vi "FileCreatorMain.vi"() -> ()   [LabVIEW 2017]
uses:
  AutoFileDataType.ctl
panel:
  in  "Flip This Auto":bool
  in  "Auto":T1
  in  "Path File Name":string[](array[string])
  out "standard output":string
  out "standard error":string="NI Linux Real-Time (run mode)\n\nLog in with your NI-Auth credentials.\n\n"
  in  "ExportAllToRobot":bool
  in  "SaveToLocal":bool
  in  "LoadFromLocal":bool
  in  "ExportToRobot":bool
  in  "LoadAllFromRobot":bool
  in  "LocalFiles":i32(listbox)=2
  in  "LocalFileNames":string[](array[string])=["1A.txt", "1B.txt", "1C.txt", "1D.txt", "2A.txt", "2B.txt", "2C.txt", "2D.txt", "3A.txt", "3B.txt", "3C.txt", "3D.txt", "4A.txt", "4B.txt", "4C.txt", "4D.txt"]
  # "Drive:\nWait or\nStart"
  # "Elevator:\nWait or\nStart"
  # "Intake:\nWait or\nStart"
  # "Distance \nfor\nElevator"
  # "Degrees \nto turn"
  # "Elevator\nCommand"
  # "Time for \nintake"
  # "Drive\ncommand"
  # "Time\nfor elevator"
  # "Elevator\n Speed"
  # "Intake \nCommand"
  # "Path File Path"
  # "Speed"
  # "Distance(in)"
  # "Intake Speed"
  # "Drive commands:\n1. For time\n2. For distance\n3. Turn for angle\n4. Stop\n5. Drive Path\n6. Turn To Angle\n7. Drive to Cube"
  # "Elevator Commands:\n1. For time\n2. To distance\n3. Stop\n4. Pause for time, then distance"
  # "Intake Commands:\n1. For time\n2. Until cube\n3. Stop"
  # "Wait: 0\nStart: 1"
  # "Responses of CMDs run"
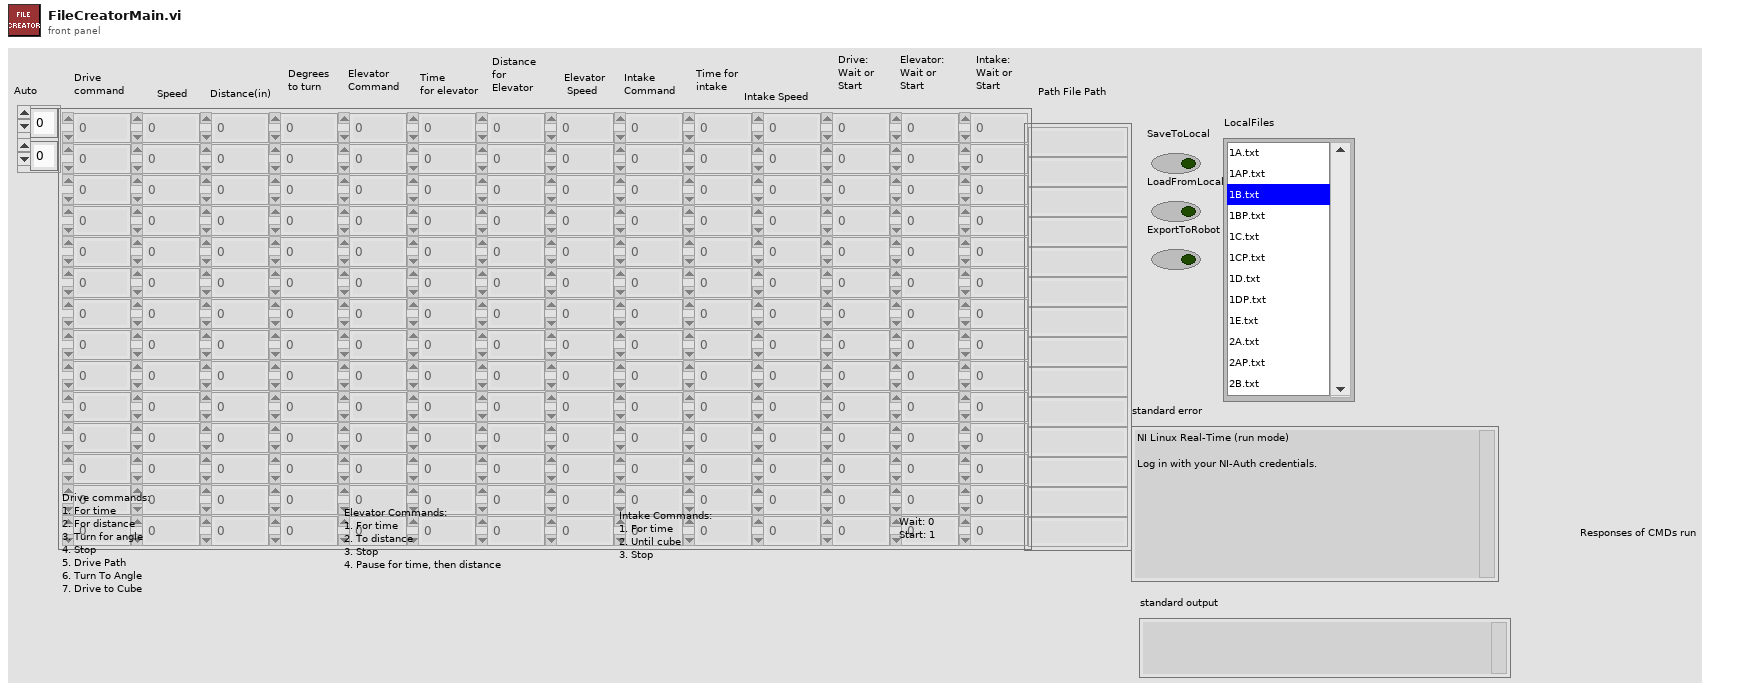
[diagram p1: front panel]
types:
  T1 = typedef "AutoFileDataType.ctl" = dbl[][]
  T2 = enum16{"open", "replace", "create", "open or create", "replace or create", "replace or create with confirmation"}
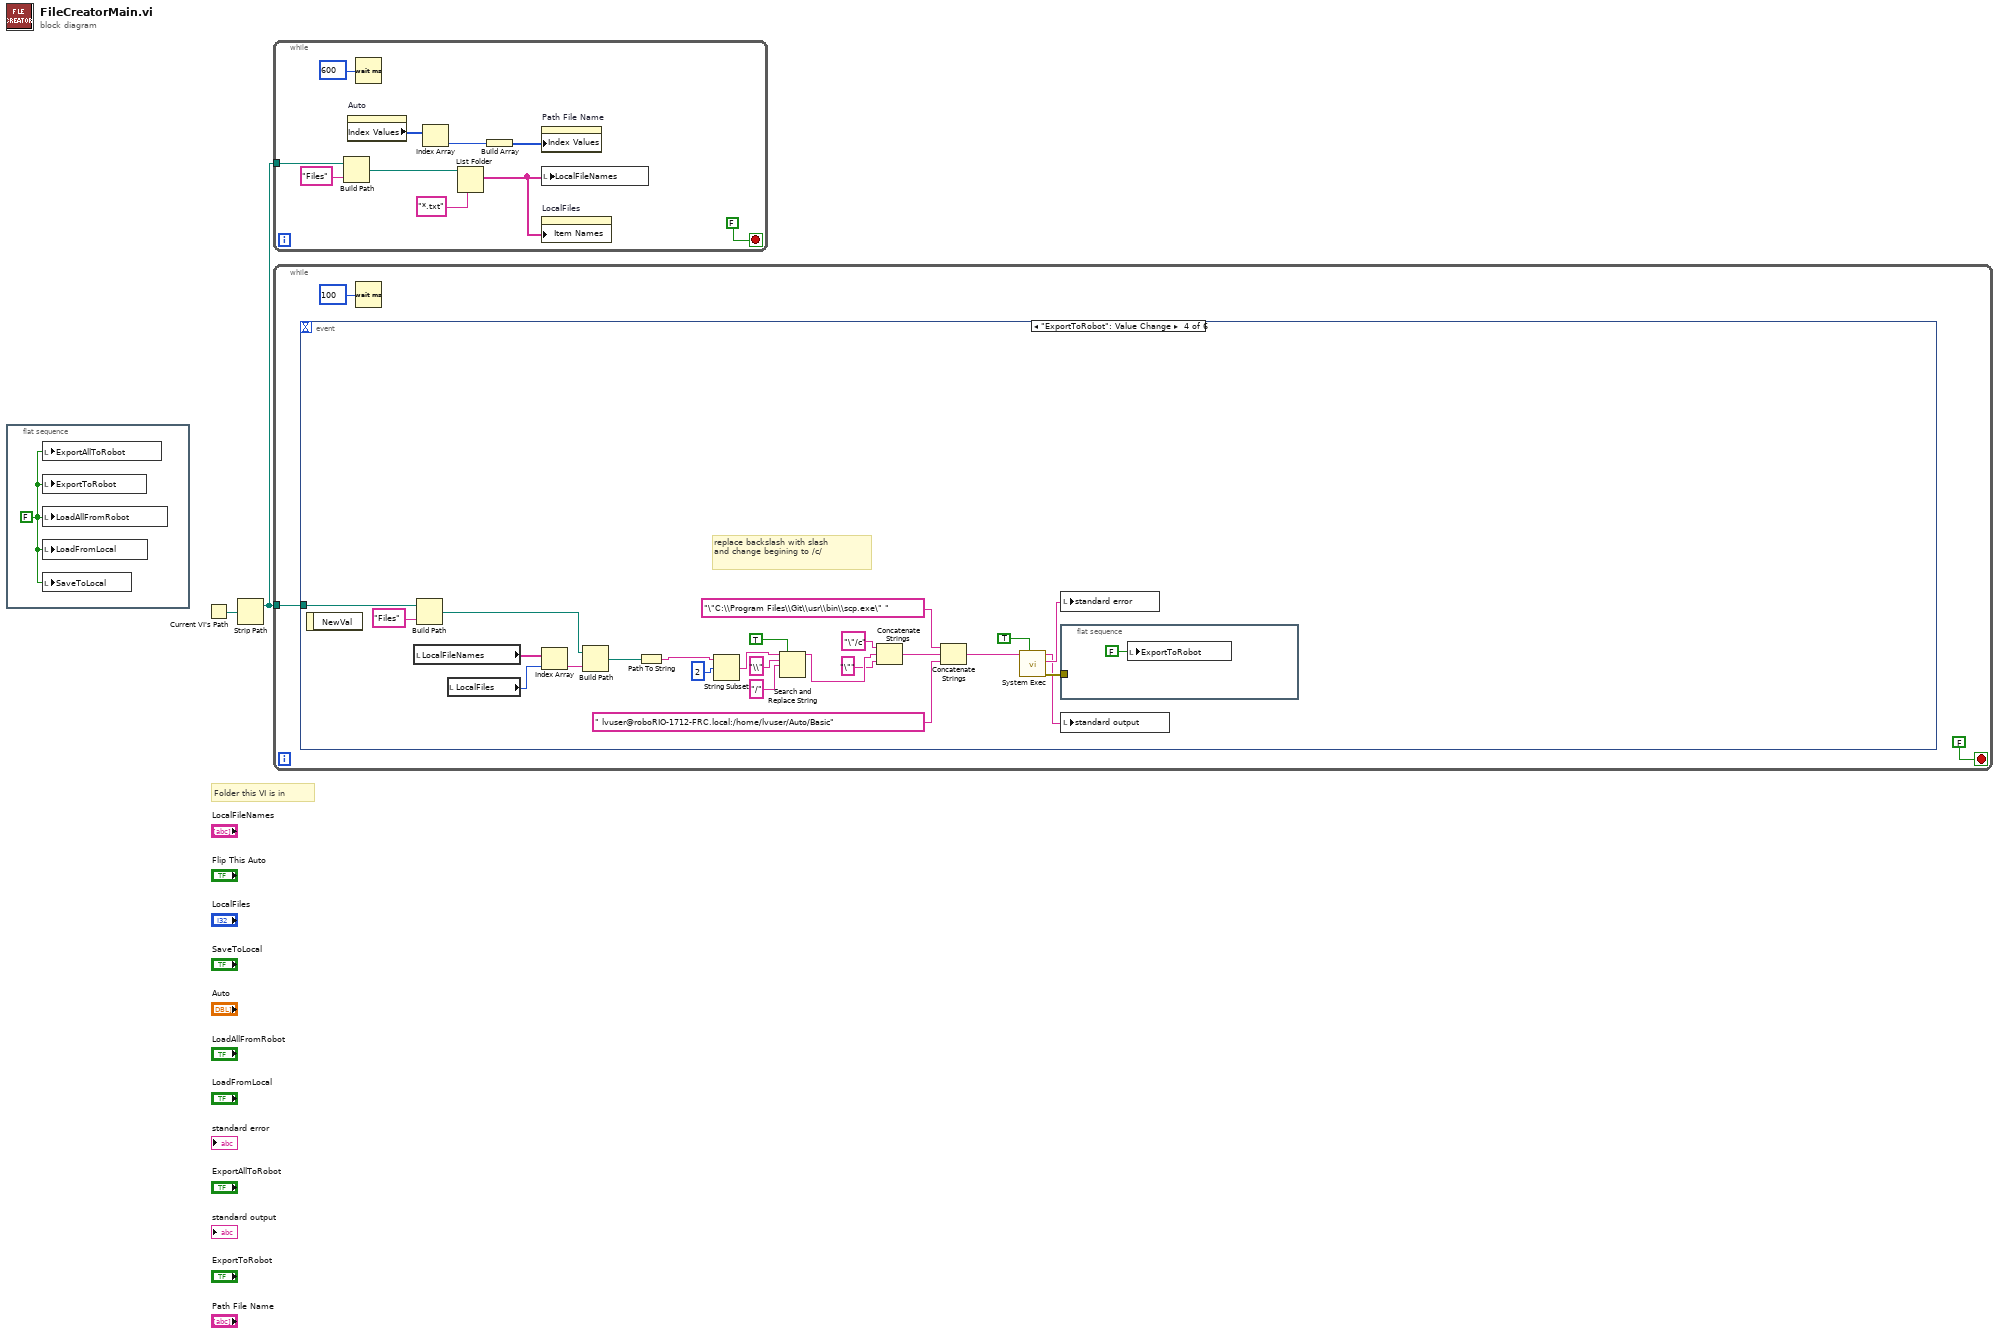
[diagram p0: block diagram]
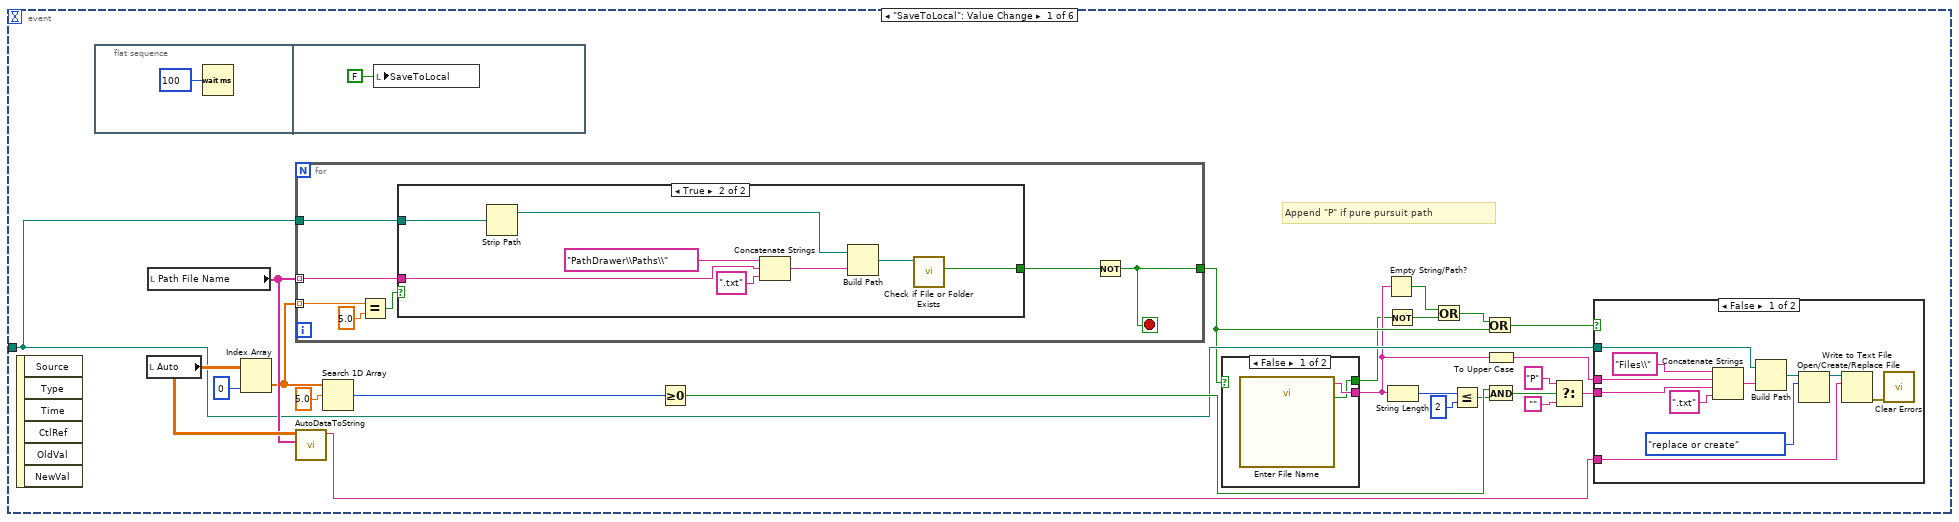
[diagram p2: hidden frame]
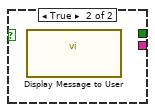
[diagram p3: hidden frame]
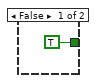
[diagram p4: hidden frame]
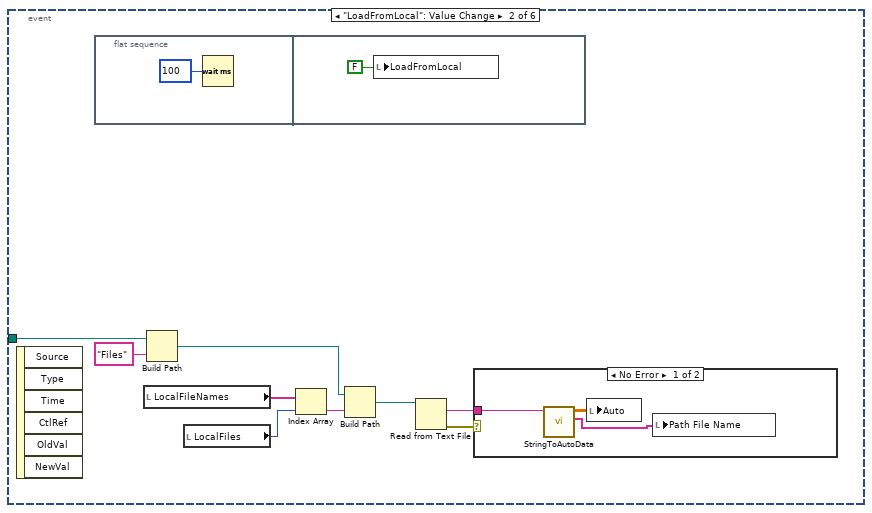
[diagram p6: hidden frame]
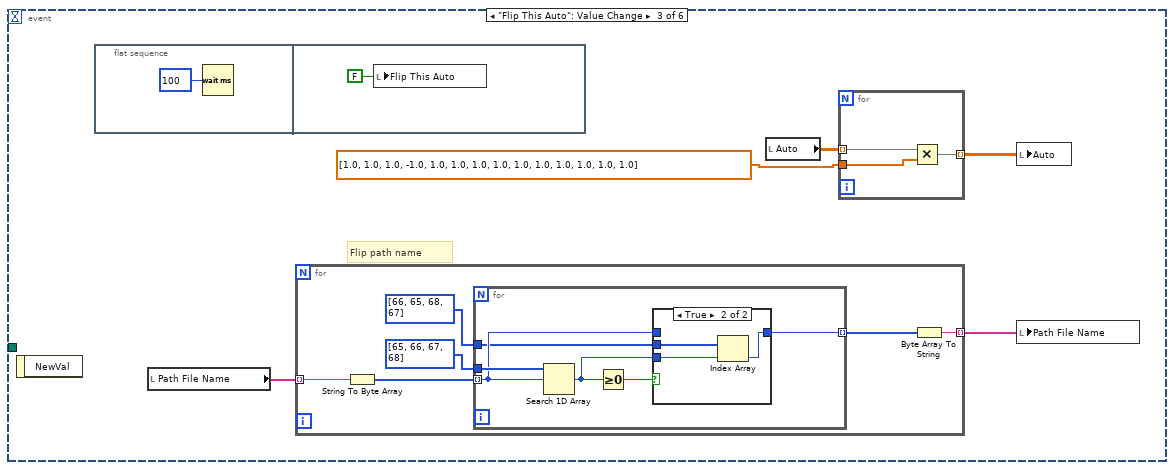
[diagram p8: hidden frame]
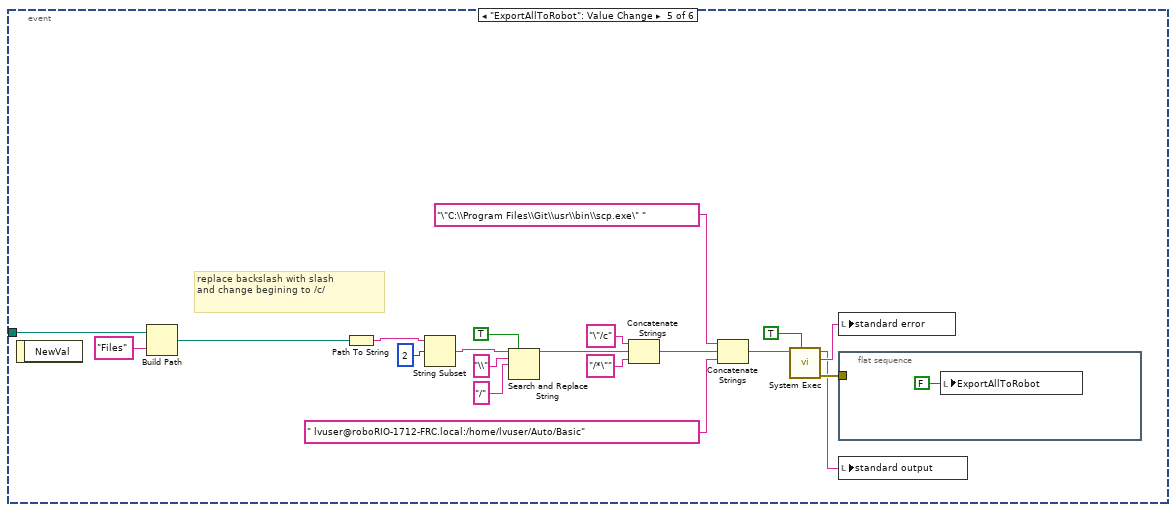
[diagram p10: hidden frame]
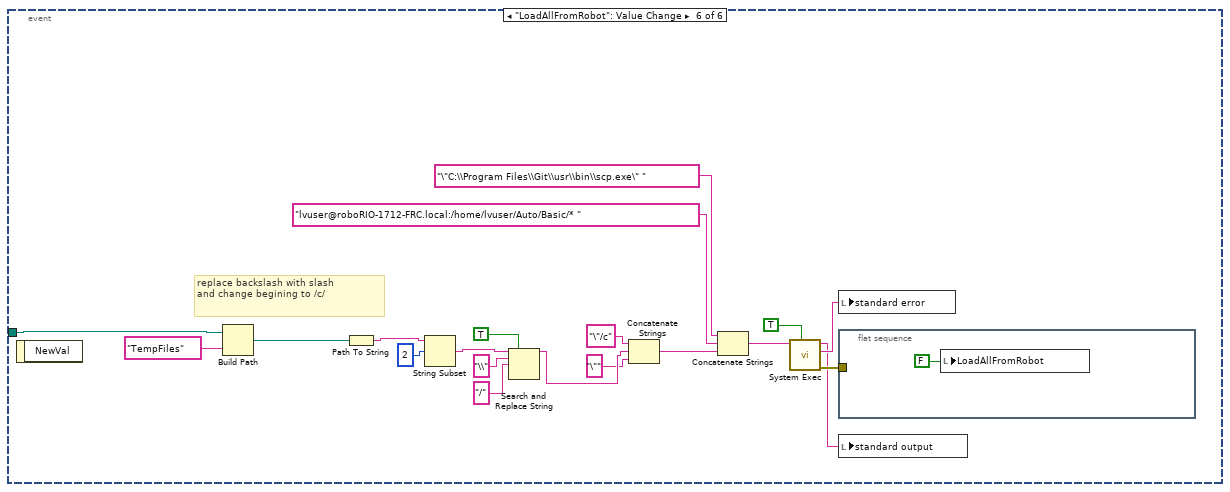
[diagram p11: hidden frame]
diagram:
  # "Folder this VI is in"
  n1 = flat-sequence {
    frame #0 {
      w3 = FALSE ("ExportToRobot")
      n2 = local write "ExportAllToRobot"(w3) -> ()
      n3 = local write "ExportToRobot"(w3) -> ()
      n4 = local write "LoadAllFromRobot"(w3) -> ()
      n5 = local write "LoadFromLocal"(w3) -> ()
      n6 = local write "SaveToLocal"(w3) -> ()
    }
  }
  n7 = Current VI's Path() -> (path=w2:path)
  n8 = Strip Path(path=w2) -> (stripped path=w1:path)  [unwired: 1 out]
  n9 = while {
    tunnel: w1 -> [w9]
    stop <- FALSE stop-if-true
    n10 = Build Path(base path=w9, name or relative path="Files") -> (appended path=w11:path)
    n11 = property on="Auto" class="Arr (strict)"() -> ("Index Values"=w6:u32[])  [unwired: 2 in, 2 out]
    n12 = Wait (ms)(milliseconds to wait=u32 600) -> ()  [unwired: 1 out]
    n13 = Index Array(array=w6) -> (element=w5:u32)  [unwired: 1 in]
    n14 = List Folder(path=w11, pattern="*.txt") -> (filenames=w7:string[])  [unwired: 2 in, 3 out]
    n15 = Build Array(w5) -> (w4:u32[])
    n16 = property on="Path File Name" class="Arr (strict)"("Index Values"=w4) -> ()  [unwired: 2 in, 2 out]
    n17 = local write "LocalFileNames"(w7) -> ()
    n18 = property on="LocalFiles" class="LstBox (strict)"("Item Names"=w7) -> ()  [unwired: 2 in, 2 out]
  }
  n19 = while {
    tunnel: w1 -> [w15]
    stop <- FALSE stop-if-true
    n20 = event shown="[3] \"ExportToRobot\": Value Change" {
      selector: _ -> [_ _ _ _ _ _]
      dyn-events: _ -> [_ _ _ _ _ _]
      timeout: _ -> [_ _ _ _ _ _]
      tunnel: w15 -> [w23 w76 _ w130 w155 w176]
      event "SaveToLocal": Value Change {
        # "Append \"P\" if pure pursuit path"
        n21 = event-data() -> ()  [unwired: 1 in, 6 out]
        n22 = flat-sequence {
          frame #0 {
            n23 = Wait (ms)(milliseconds to wait=u32 100) -> ()  [unwired: 1 out]
          }
          frame #1 {
            n24 = local write "SaveToLocal"(FALSE ("SaveToLocal")) -> ()
          }
        }
        n25 = local read "Auto"() -> (w25:T1)
        n26 = local read "Path File Name"() -> (w24:string[])
        n27 = Index Array(array=w25, index (col)=0 ("disabled index (col)")) -> (element=w22:dbl[])  [unwired: 1 in]
        n28 = for {
          tunnel: w24 -> [w47] mode=indexing
          tunnel: w23 -> [w46]
          tunnel: w22 -> [w45] mode=indexing
          tunnel: [w43] -> w19
          stop <- w43 stop-if-true
          n29 = Equal?(x=w45, y=5.0) -> (x = y?=w48:bool)
          n30 = case shown="True" w48 {
            tunnel: w47 -> [_ w53]
            tunnel: w46 -> [_ w58]
            tunnel: [TRUE ("file or folder exists?") w56] -> w44
            frame False {
            }
            frame True {
              n31 = Strip Path(path=w58) -> (stripped path=w55:path)  [unwired: 1 out]
              n32 = Concatenate Strings("PathDrawer\\Paths\\" ("name or relative path"), w53, ".txt" ("string")) -> (w51:string)
              n33 = Build Path(base path=w55, name or relative path=w51) -> (appended path=w57:path)
              n34 = call <vilib>:"Check if File or Folder Exists.vi"("path"=w57) -> ("file or folder exists?"=w56:bool)  [unwired: 8 in, 2 out]
            }
          }
          n35 = Not(x=w44) -> (.not. x?=w43:bool)
        }
        n36 = call "AutoDataToString.vi"("File Path Name"=w24, "Auto"=w25) -> ("String"=w37:string)  [unwired: 9 in]
        n37 = Search 1D Array(1D array=w22, element=5.0) -> (index of element=w35:i32)  [unwired: 1 in]
        n38 = Greater Or Equal To 0?(x=w35) -> (x >= 0?=w30:bool)
        n39 = case shown="False" w19 {
          tunnel: [w42 _] -> w18
          tunnel: [w41 _] -> w17
          frame False {
            n40 = call "Enter File Name"() -> ("File Name"=w42:string, "Enter"=w41:bool)  [unwired: 17 in, 1 out]
          }
          frame True {
            n41 = call "Display Message to User"() -> ()  [unwired: 10 in, 2 out]
          }
        }
        n42 = Empty String/Path?(string/path=w18) -> (empty?=w40:bool)
        n43 = Not(x=w17) -> (.not. x?=w39:bool)
        n44 = String Length(string=w18) -> (length=w29:i32)
        n45 = Or(x=w40, y=w39) -> (x .or. y?=w21:bool)
        n46 = Less Or Equal?(x=w29, y=2) -> (x <= y?=w27:bool)
        n47 = Or(x=w21, y=w19) -> (x .or. y?=w20:bool)
        n48 = To Upper Case(1:w18) -> (0:w38:string)
        n49 = And(x=w30, y=w27) -> (x .and. y?=w26:bool)
        n50 = Select(t="P", s=w26, f="") -> (s? t:f=w32:string)
        n51 = case shown="False" w20 {
          tunnel: w38 -> [w68 _]
          tunnel: w37 -> [w67 _]
          tunnel: w23 -> [w63 _]
          tunnel: w32 -> [w61 _]
          frame False {
            n52 = Concatenate Strings("Files\\" ("name or relative path"), w68, w61, ".txt" ("string")) -> (w71:string)
            n53 = Build Path(base path=w63, name or relative path=w71) -> (appended path=w66:path)
            n54 = Open/Create/Replace File(file path (use dialog)=w66, operation (0:open)=T2."replace or create") -> (refnum out=w65:refnum<file>)  [unwired: 4 in, 2 out]
            n55 = Write to Text File(file (use dialog)=w65, text=w67) -> (error out=w69:errorcluster)  [unwired: 2 in, 2 out]
            n56 = call <vilib>:"Clear Errors.vi"("error in (no error)"=w69) -> ()  [unwired: 5 in, 2 out]
          }
          frame True {
          }
        }
      }
      event "LoadFromLocal": Value Change {
        n57 = event-data() -> ()  [unwired: 1 in, 6 out]
        n58 = flat-sequence {
          frame #0 {
            n59 = Wait (ms)(milliseconds to wait=u32 100) -> ()  [unwired: 1 out]
          }
          frame #1 {
            n60 = local write "LoadFromLocal"(FALSE ("SaveToLocal")) -> ()
          }
        }
        n61 = local read "LocalFileNames"() -> (w75:string[])
        n62 = Build Path(base path=w76, name or relative path="Files") -> (appended path=w79:path)
        n63 = local read "LocalFiles"() -> (w74:i32)
        n64 = Index Array(array=w75, index=w74) -> (element=w78:string)
        n65 = Build Path(base path=w79, name or relative path=w78) -> (appended path=w77:path)
        n66 = Read from Text File(file (use dialog)=w77) -> (text=w72:string, error out=w73:errorcluster)  [unwired: 3 in, 2 out]
        n67 = case shown="No Error" w73 {
          tunnel: w72 -> [w85 _]
          frame No Error {
            n68 = call "StringToAutoData.vi"("String"=w85) -> ("Path File Names"=w83:string[], "Auto"=w84:T1)  [unwired: 9 in]
            n69 = local write "Auto"(w84) -> ()
            n70 = local write "Path File Name"(w83) -> ()
          }
          frame Error {
          }
        }
      }
      event "Flip This Auto": Value Change {
        # "Flip path name"
        n71 = event-data() -> ()  [unwired: 1 in, 1 out]
        n72 = flat-sequence {
          frame #0 {
            n73 = Wait (ms)(milliseconds to wait=u32 100) -> ()  [unwired: 1 out]
          }
          frame #1 {
            n74 = local write "Flip This Auto"(FALSE ("Flip This Auto")) -> ()
          }
        }
        n75 = local read "Path File Name"() -> (w87:string[])
        n76 = for {
          tunnel: w87 -> [w94] mode=indexing
          tunnel: [w92] -> w86 mode=indexing
          n77 = String To Byte Array(string=w94) -> (unsigned byte array=w96:u8[])
          n78 = for {
            tunnel: w96 -> [w99] mode=indexing
            tunnel: u8[] [65, 66, 67, 68] ("1D array") -> [w102]
            tunnel: [w100] -> w93 mode=indexing
            tunnel: u8[] [66, 65, 68, 67] ("1D array") -> [w97]
            n79 = Search 1D Array(1D array=w102, element=w99) -> (index of element=w98:i32)  [unwired: 1 in]
            n80 = Greater Or Equal To 0?(x=w98) -> (x >= 0?=w101:bool)
            n81 = case shown="True" w101 {
              tunnel: [w103 w106] -> w100
              tunnel: w99 -> [w103 _]
              tunnel: w98 -> [_ w105]
              tunnel: w97 -> [_ w104]
              frame False {
              }
              frame True {
                n82 = Index Array(array=w104, index=w105) -> (element=w106:u8)
              }
            }
          }
          n83 = Byte Array To String(unsigned byte array=w93) -> (string=w92:string)
        }
        n84 = local read "Auto"() -> (w89:T1)
        n85 = for {
          tunnel: dbl[] [1.0, 1.0, 1.0, -1.0, 1.0, 1.0, 1.0, 1.0, 1.0, 1.0, 1.0, 1.0, 1.0, 1.0] -> [w111]
          tunnel: w89 -> [w110] mode=indexing
          tunnel: [w109] -> w88 mode=indexing
          n86 = Multiply(x=w110, y=w111) -> (x*y=w109:dbl[])
        }
        n87 = local write "Auto"(w88) -> ()
        n88 = local write "Path File Name"(w86) -> ()
      }
      event "ExportToRobot": Value Change {
        # "replace backslash with slash\nand change begining to /c/"
        n89 = event-data() -> ()  [unwired: 1 in, 1 out]
        n90 = local read "LocalFileNames"() -> (w133:string[])
        n91 = Build Path(base path=w130, name or relative path="Files") -> (appended path=w135:path)
        n92 = local read "LocalFiles"() -> (w132:i32)
        n93 = Index Array(array=w133, index=w132) -> (element=w134:string)
        n94 = Build Path(base path=w135, name or relative path=w134) -> (appended path=w114:path)
        n95 = Path To String(path=w114) -> (string=w122:string)
        n96 = String Subset(string=w122, offset (0)=2) -> (substring=w120:string)  [unwired: 1 in]
        n97 = Search and Replace String(replace all?=TRUE ("replace all? (F)"), input string=w120, search string="\\", replace string="/" ("replace string (\"\")")) -> (result string=w119:string)  [unwired: 4 in, 3 out]
        n98 = Concatenate Strings("\"/c" ("string"), w119, "\"" ("string")) -> (w117:string)
        n99 = Concatenate Strings("\"C:\\Program Files\\Git\\usr\\bin\\scp.exe\" " ("command line"), w117, " lvuser@roboRIO-1712-FRC.local:/home/lvuser/Auto/Basic" ("string")) -> (w126:string)
        n100 = call <vilib>:"System Exec.vi"("wait until completion? (T)"=TRUE, "command line"=w126) -> ("error out"=w115:errorcluster, "standard error"=w113:string, "standard output"=w112:string)  [unwired: 6 in, 1 out]
        n101 = local write "standard error"(w113) -> ()
        n102 = flat-sequence {
          tunnel: w115 -> [_]
          frame #0 {
            n103 = local write "ExportToRobot"(FALSE ("Export To File")) -> ()
          }
        }
        n104 = local write "standard output"(w112) -> ()
      }
      event "ExportAllToRobot": Value Change {
        # "replace backslash with slash\nand change begining to /c/"
        n105 = event-data() -> ()  [unwired: 1 in, 1 out]
        n106 = Build Path(base path=w155, name or relative path="Files") -> (appended path=w137:path)
        n107 = Path To String(path=w137) -> (string=w147:string)
        n108 = String Subset(string=w147, offset (0)=2) -> (substring=w145:string)  [unwired: 1 in]
        n109 = Search and Replace String(replace all?=TRUE ("replace all? (F)"), input string=w145, search string="\\", replace string="/" ("replace string (\"\")")) -> (result string=w144:string)  [unwired: 4 in, 3 out]
        n110 = Concatenate Strings("\"/c" ("string"), w144, "/*\"" ("string")) -> (w142:string)
        n111 = Concatenate Strings("\"C:\\Program Files\\Git\\usr\\bin\\scp.exe\" " ("command line"), w142, " lvuser@roboRIO-1712-FRC.local:/home/lvuser/Auto/Basic" ("string")) -> (w151:string)
        n112 = call <vilib>:"System Exec.vi"("wait until completion? (T)"=TRUE, "command line"=w151) -> ("error out"=w140:errorcluster, "standard error"=w139:string, "standard output"=w138:string)  [unwired: 6 in, 1 out]
        n113 = local write "standard error"(w139) -> ()
        n114 = flat-sequence {
          tunnel: w140 -> [_]
          frame #0 {
            n115 = local write "ExportAllToRobot"(FALSE ("Export To File")) -> ()
          }
        }
        n116 = local write "standard output"(w138) -> ()
      }
      event "LoadAllFromRobot": Value Change {
        # "replace backslash with slash\nand change begining to /c/"
        n117 = event-data() -> ()  [unwired: 1 in, 1 out]
        n118 = Build Path(base path=w176, name or relative path="TempFiles") -> (appended path=w160:path)
        n119 = Path To String(path=w160) -> (string=w169:string)
        n120 = String Subset(string=w169, offset (0)=2) -> (substring=w167:string)  [unwired: 1 in]
        n121 = Search and Replace String(replace all?=TRUE ("replace all? (F)"), input string=w167, search string="\\", replace string="/" ("replace string (\"\")")) -> (result string=w166:string)  [unwired: 4 in, 3 out]
        n122 = Concatenate Strings("\"/c" ("string"), w166, "\"" ("string")) -> (w158:string)
        n123 = Concatenate Strings("\"C:\\Program Files\\Git\\usr\\bin\\scp.exe\" " ("command line"), "lvuser@roboRIO-1712-FRC.local:/home/lvuser/Auto/Basic/* " ("string"), w158) -> (w173:string)
        n124 = call <vilib>:"System Exec.vi"("wait until completion? (T)"=TRUE, "command line"=w173) -> ("error out"=w163:errorcluster, "standard error"=w162:string, "standard output"=w161:string)  [unwired: 6 in, 1 out]
        n125 = local write "standard error"(w162) -> ()
        n126 = flat-sequence {
          tunnel: w163 -> [_]
          frame #0 {
            n127 = local write "LoadAllFromRobot"(FALSE ("Export To File")) -> ()
          }
        }
        n128 = local write "standard output"(w161) -> ()
      }
    }
    n129 = Wait (ms)(milliseconds to wait=u32 100) -> ()  [unwired: 1 out]
  }
